vi "currentmeasure__9fa348117f.vi"() -> ()   [LabVIEW 2023]
uses:
  <instrlib>/niDCPower/nidcpower.llb/niDCPower Auto Zero.ctl
  <vilib>/Utility/error.llb/DialogType.ctl
  <instrlib>/niDCPower/nidcpower.llb/niDCPower Aperture Time Units.ctl
  <vilib>/DAQmx/read.llb/DAQmx Read (Analog 1D DBL 1Chan NSamp).vi
  <vilib>/DAQmx/create/channels.llb/DAQmx Create Channel (AI-Voltage-Basic).vi
  <vilib>/DAQmx/configure/timing.llb/DAQmx Timing (Sample Clock).vi
  <vilib>/DAQmx/configure/task.llb/DAQmx Configure Logging (TDMS).vi
  <vilib>/DAQmx/configure/trigger.llb/DAQmx Start Trigger (Digital Edge).vi
  <vilib>/DAQmx/miscellaneous.llb/DAQmx Fill In Error Info.vi
  <resource>/objmgr/daqmx.rc
panel:
  out "Waveform Graph 3":dynamicdata(graph)
  out "Waveform Graph 2":dbl[](graph)
  in  "Trigger Type":T1(tab)
  out "Waveform Graph":dbl[](graph)
  in  "Stop":bool
  in  "Number of Samples":i32=100
  in  "TDMS File Path":path
  in  "Sample Rate":dbl=1000.0
  in  "Sample Clock Source":tag="OnboardClock"
  in  "Terminal Configuration":i32(ring)=-1 items=["default"=-1, "RSE"=10083, "NRSE"=10078, "Differential"=10106, "Pseudodifferential"=12529]
  in  "Max Voltage":dbl=5.0
  in  "Min Voltage":dbl=-5.0
  in  "Physical Channel":tag="Dev1/ai0"
  out "Actual Sample Rate":dbl=1000.0 format="%0.2f"
  in  "Logging Mode":i32(ring)=10231 items=["Off"=10231, "Log and Read"=15842]
  in  "Auto Zero":T2 items=["Off"=0, "Once"=1024, "On"=1]
  in  "Measure Record Length Is Finite":bool=TRUE caption="Measure Record Length \nIs Finite"
  in  "Samples to Average":i32=1
  in  "Measure Record Length 2":i32=100 caption="Measure Record Length"
  out "Effective Measurement Rate":dbl
  in  "Voltage Level":dbl=5.0 format="%.4p"
  in  "Channel Name":string="0"
  in  "Resource Name":refnum<k15>="Dev1"
  # "To enable triggers, select a tab above, and configure the settings.\n\nNot all hardware supports all trigger types. Refer to your device documentation for more information."
  # "This trigger type is not supported in continuous sample timing. \n\nRefer to your device documentation for more information on which triggers are supported."
  # "This trigger type is not supported in continuous sample timing. \n\nRefer to your device documentation for more information on which triggers are supported."
  # "If time is not manually set, task will begin after 10 seconds"
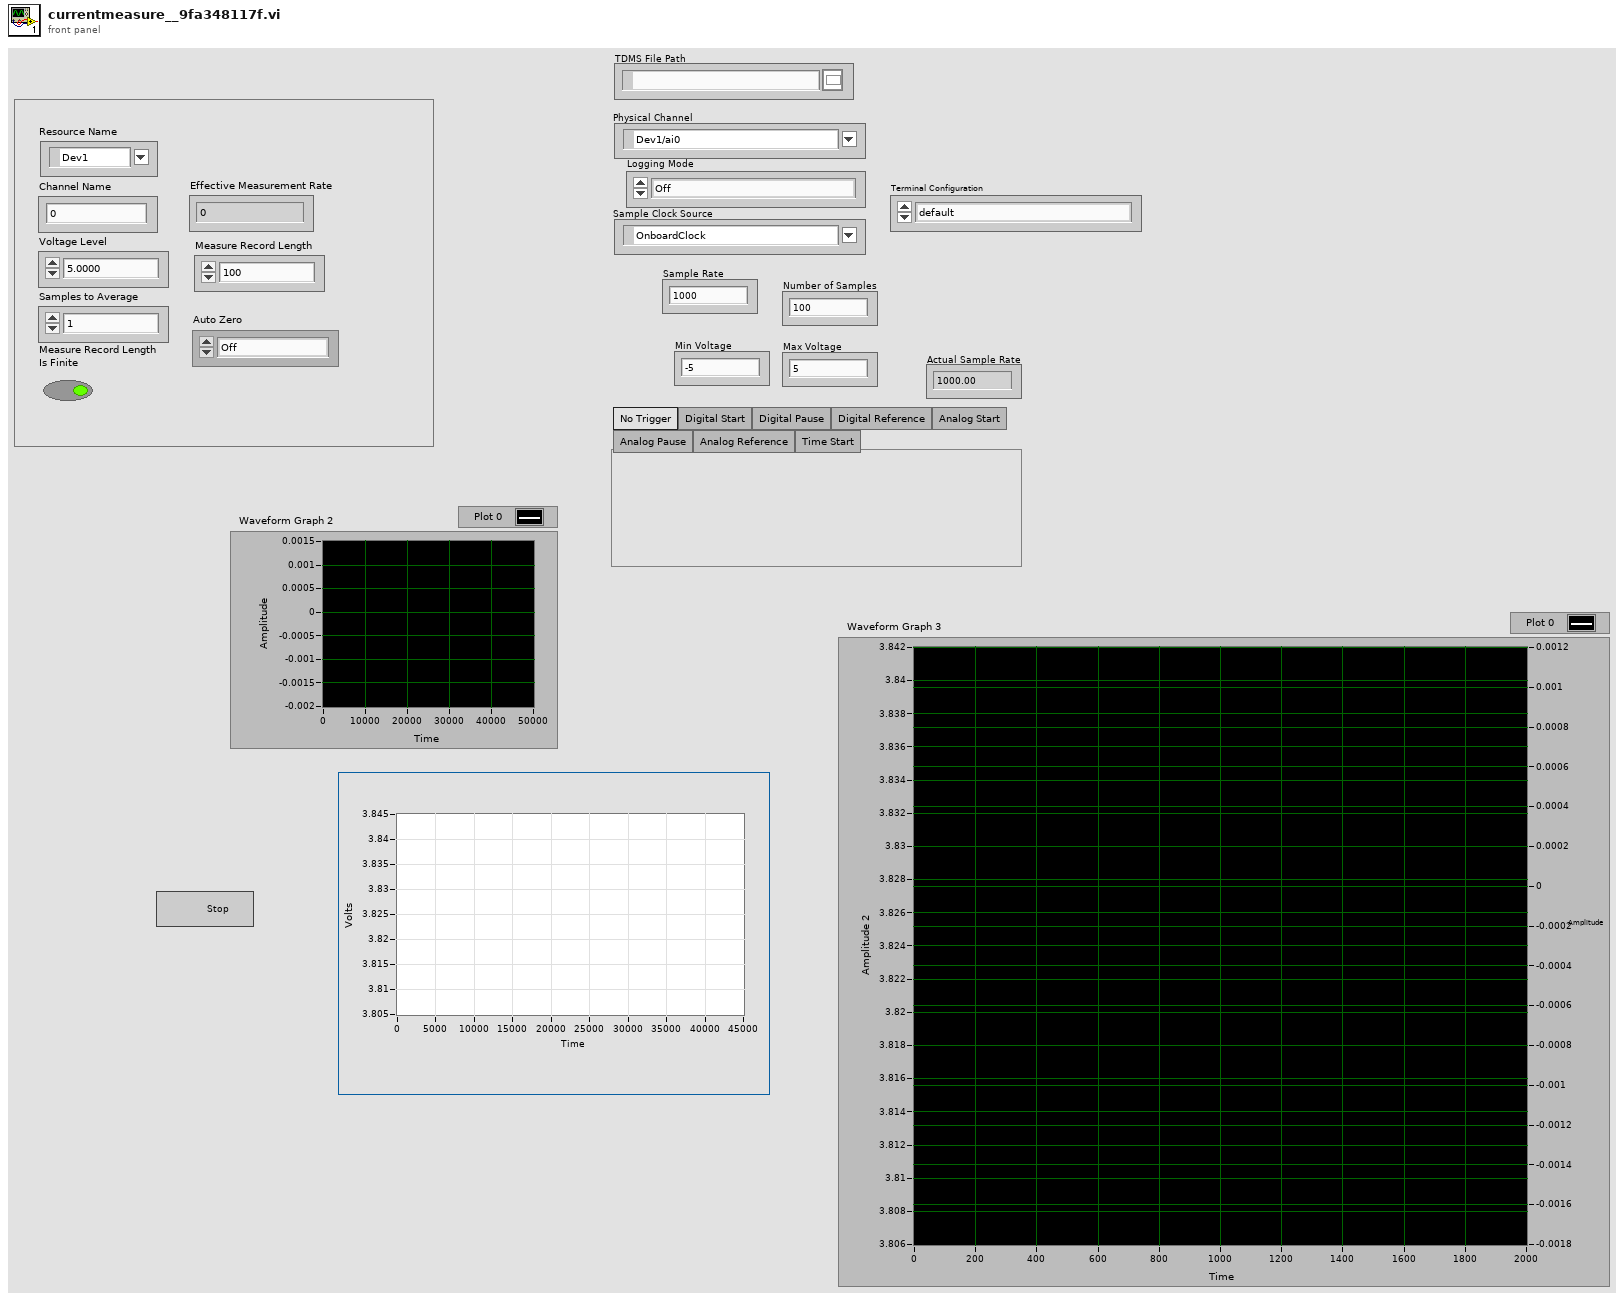
[diagram p1: front panel]
types:
  T1 = enum32{"No Trigger", "Digital Start", "Digital Pause", "Digital Reference", "Analog Start", "Analog Pause", "Analog Reference", "Time Start"}
  T2 = typedef "niDCPower Auto Zero.ctl" = i32
  T3 = typedef "DialogType.ctl" = u16
  T4 = typedef "niDCPower Aperture Time Units.ctl" = i32
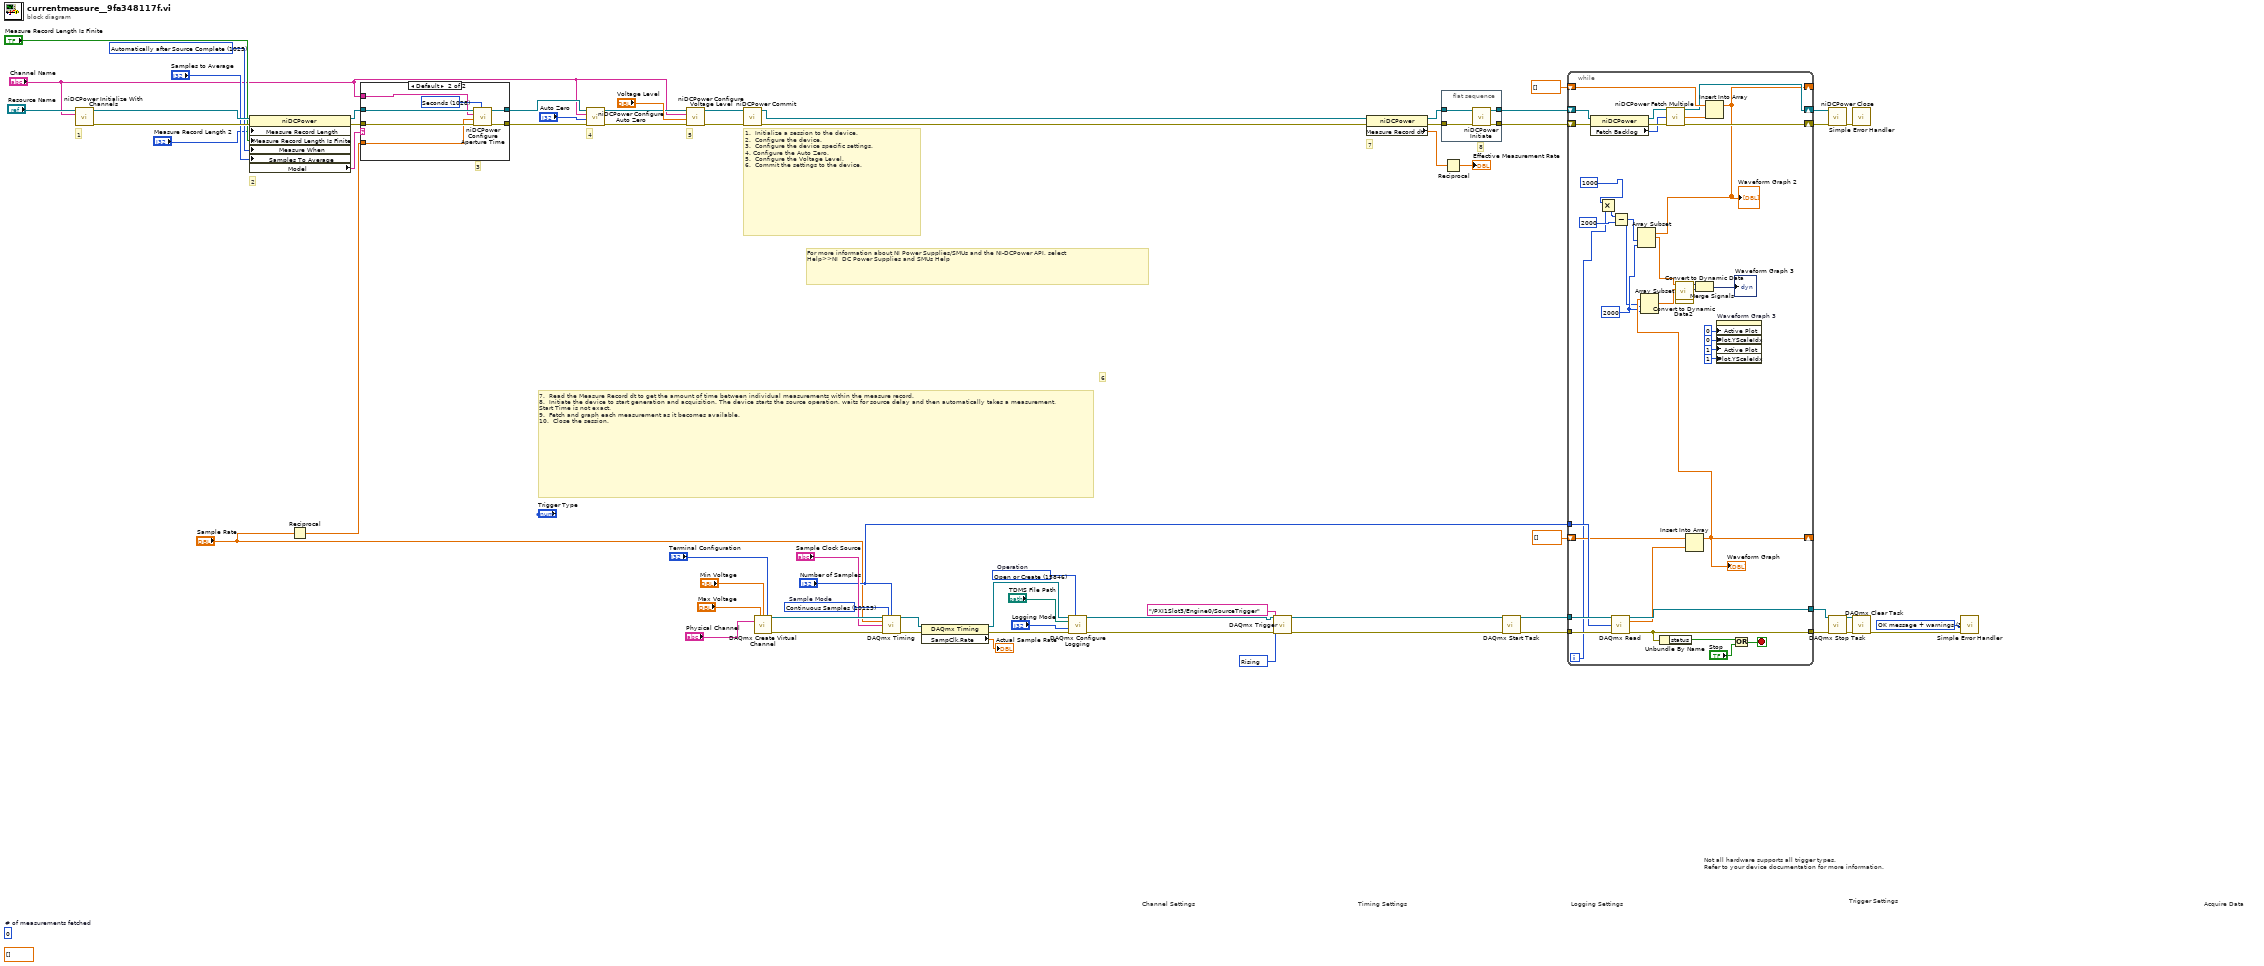
[diagram p0: block diagram]
diagram:
  w3 = 10280 items=["Rising"=10280, "Falling"=10171] ("edge")
  w19 = T3 3 items=["no dialog", "OK message", "continue or stop message", "OK message + warnings", "continue/stop + warnings"] ("type of dialog (OK msg:1)")
  w36 = 15846 items=["Open"=10437, "Open or Create"=15846, "Create or Replace"=15847, "Create"=15848]  # Operation
  w41 = 10123 items=["Finite Samples"=10178, "Continuous Samples"=10123, "Hardware Timed Single Point"=12522]  # Sample Mode
  (unwired) dbl[] []
  (unwired) 0  # # of measurements fetched
  w62 = 1025 items=["Automatically after Source Complete"=1025, "On Demand"=1026, "On Measure Trigger"=1027] ("Measurement:Advanced:Measure When")
  # "Trigger Settings"
  # "Not all hardware supports all trigger types.\nRefer to your device documentation for more information."
  # "Acquire Data"
  # "Timing Settings"
  # "Channel Settings"
  # "Logging Settings"
  # "7.  Read the Measure Record dt to get the amount of time between individual measurements within the measure record.\n8.  Initiate the device to start generation and acquisition. The device starts the source operation, waits for source delay and then automatically takes a measurement.\nStart Time is not exact.\n9.  Fetch and graph each measurement as it becomes available.\n10.  Close the session."
  # "8"
  # "7"
  # "6"
  # "5"
  # "4"
  # "2"
  # "1"
  # "1.  Initialize a session to the device.\n2.  Configure the device.\n3.  Configure the device specific settings.\n4. Configure the Auto Zero.\n5.  Configure the Voltage Level.\n6.  Commit the settings to the device."
  # "3"
  # "For more information about NI Power Supplies/SMUs and the NI-DCPower API, select\nHelp>>NI  DC Power Supplies and SMUs Help"
  n1 = call <instrlib>:"niDCPower Initialize With Channels.vi"("channels"="Channel Name", "resource name"="Resource Name") -> ("error out"=w63:errorcluster, "instrument handle out"=w64:refnum<k15>)  [unwired: 3 in, 5 out]
  n2 = property class="niDCPower"(reference=w64, error in=w63, "Measure Record Length"="Measure Record Length 2", "Measure Record Length Is Finite"="Measure Record Length Is Finite", "Measure When"=w62, "Samples To Average"="Samples to Average") -> (reference out=w53:refnum<k15>, error out=w52:errorcluster, "Model"=w54:string)
  n3 = Reciprocal(x="Sample Rate") -> (1/x=w17:dbl)
  n4 = case shown="Default" w54 {
    tunnel: w53 -> [w67 w74]
    tunnel: w52 -> [w66 w73]
    tunnel: [w66 w71] -> w50
    tunnel: [w67 w70] -> w51
    tunnel: "Channel Name" -> [_ w69]
    tunnel: w17 -> [_ w68]
    frame "NI PXI-4110", "NI PXI-4130", "NI PXI-4131A", "NI PXIe-4154" {
    }
    frame Default {
      w72 = T4 1028 items=["Seconds"=1028, "Powerline Cycles"=1029] ("aperture time units")
      n5 = call <instrlib>:"niDCPower Configure Aperture Time.vi"("aperture time units"=w72, "error in (no error)"=w73, "aperture time"=w68, "channel name"=w69, "instrument handle"=w74) -> ("error out"=w71:errorcluster, "instrument handle out"=w70:refnum<k15>)  [unwired: 5 out]
    }
  }
  n6 = call <instrlib>:"niDCPower Configure Auto Zero.vi"("error in (no error)"=w50, "auto zero"="Auto Zero", "channel name"="Channel Name", "instrument handle"=w51) -> ("error out"=w48:errorcluster, "instrument handle out"=w47:refnum<k15>)  [unwired: 6 out]
  n7 = call <instrlib>:"niDCPower Configure Voltage Level.vi"("error in (no error)"=w48, "voltage level"="Voltage Level", "channel name"="Channel Name", "instrument handle"=w47) -> ("error out"=w60:errorcluster, "instrument handle out"=w59:refnum<k15>)  [unwired: 6 out]
  n8 = call <instrlib>:"niDCPower Commit.vi"("error in (no error)"=w60, "instrument handle"=w59) -> ("error out"=w1:errorcluster, "instrument handle out"=w2:refnum<k15>)  [unwired: 8 out]
  n9 = call-poly <vilib>:"DAQmx Create Virtual Channel.vi"("maximum value"="Max Voltage", "minimum value"="Min Voltage", "input terminal configuration"="Terminal Configuration", "physical channels"="Physical Channel") -> ("task out"=w39:refnum<k21>, "error out"=w40:errorcluster)  [unwired: 10 in]
  n10 = call-poly <vilib>:"DAQmx Timing.vi"("task/channels in"=w39, "sample mode"=w41, "samples per channel"="Number of Samples", "rate"="Sample Rate", "source"="Sample Clock Source", "error in"=w40) -> ("task out"=w43:refnum<k21>, "error out"=w42:errorcluster)  [unwired: 8 in]
  n11 = property class="DAQmx Timing"(reference=w43, error in=w42) -> (reference out=w38:refnum<k21>, error out=w37:errorcluster, "SampClk.Rate"=→"Actual Sample Rate":dbl)
  n12 = call-poly <vilib>:"DAQmx Configure Logging.vi"("task/channels in"=w38, "operation"=w36, "file path"="TDMS File Path", "logging mode"="Logging Mode", "error in"=w37) -> ("task out"=w8:refnum<k21>, "error out"=w5:errorcluster)  [unwired: 9 in]
  n13 = call-poly <vilib>:"DAQmx Trigger.vi"("task/channels in"=w8, "source"=tag "/PXI1Slot3/Engine0/SourceTrigger", "edge"=w3, "error in"=w5) -> ("task out"=w7:refnum<k21>, "error out"=w6:errorcluster)  [unwired: 10 in]
  n14 = property class="niDCPower"(reference=w2, error in=w1) -> (reference out=w58:refnum<k15>, error out=w57:errorcluster, "Measure Record dt"=w45:dbl)
  n15 = flat-sequence {
    tunnel: [w78] -> w15
    tunnel: [w77] -> w16
    tunnel: w58 -> [w76]
    tunnel: w57 -> [w75]
    frame #0 {
      n16 = call <instrlib>:"niDCPower Initiate.vi"("error in (no error)"=w75, "instrument handle"=w76) -> ("error out"=w78:errorcluster, "instrument handle out"=w77:refnum<k15>)  [unwired: 8 out]
    }
  }
  n17 = Reciprocal(x=w45) -> (1/x=→"Effective Measurement Rate":dbl)
  n18 = call <vilib>:"DAQmx Start Task.vi"("task/channels in"=w7, "error in"=w6) -> ("task out"=w35:refnum<k21>, "error out"=w34:errorcluster)  [unwired: 12 in]
  n19 = while {
    tunnel: w35 -> [w114]
    tunnel: w34 -> [w113]
    tunnel: [w112] -> w23
    tunnel: [w110] -> w22
    tunnel: "Number of Samples" -> [w107]
    shift-right: [w88] -> _
    shift-left: dbl[] [] -> [w102]
    shift-right: [w100] -> w13
    shift-left: w16 -> [w106]
    shift-right: [w99] -> w12
    shift-left: w15 -> [w105]
    shift-right: [w87] -> _
    shift-left: dbl[] [] -> [w97]
    i -> [w82]
    stop <- w108 stop-if-true
    w83 = 2000 ("length")
    n20 = property class="niDCPower"(reference=w106, error in=w105) -> (reference out=w104:refnum<k15>, error out=w103:errorcluster, "Fetch Backlog"=w98:i32)
    n21 = Multiply(x=1000, y=w82) -> (x*y=w81:i32)
    n22 = call-poly <vilib>:"DAQmx Read.vi"("task/channels in"=w114, "number of samples per channel"=w107, "error in"=w113) -> ("task out"=w112:refnum<k21>, "data"=w96:dbl[], "error out"=w110:errorcluster)  [unwired: 10 in]
    n23 = Subtract(x=w81, y=2000) -> (x-y=w80:i32)
    n24 = Unbundle By Name(w110) -> ("status"=w109:bool)
    n25 = call <instrlib>:"niDCPower Fetch Multiple.vi"("instrument handle"=w104, "count (1)"=w98, "error in (no error)"=w103) -> ("instrument handle out"=w100:refnum<k15>, "current measurements"=w101:dbl[], "error out"=w99:errorcluster)  [unwired: 2 in, 8 out]
    n26 = Insert Into Array(array=w97, new element=w96) -> (w87:dbl[])  [unwired: 1 in]
    "Waveform Graph" <- w87
    n27 = Array Subset(array=w87, index=w80, length=w83) -> (w85:dbl[])
    n28 = call "Convert to Dynamic Data2"("Array"=w85) -> ("Dynamic Data Type"=w94:dynamicdata)  [unwired: 3 in]
    n29 = Insert Into Array(array=w102, new element=w101) -> (w88:dbl[])  [unwired: 1 in]
    "Waveform Graph 2" <- w88
    n30 = Array Subset(array=w88, index=w80, length=w83) -> (w86:dbl[])
    n31 = call "Convert to Dynamic Data"("Array"=w86) -> ("Dynamic Data Type"=w95:dynamicdata)  [unwired: 3 in]
    n32 = Merge Signals(w95, w94) -> (→"Waveform Graph 3":dynamicdata)
    n33 = property on="Waveform Graph 3" class="WFGraph (strict)"("Active Plot"=u32 0, "Plot.YScaleIdx"=u32 0 ("Plot.Y Scale Index"), "Active Plot"=u32 1, "Plot.YScaleIdx"=u32 1 ("Plot.Y Scale Index")) -> ()  [unwired: 2 in, 2 out]
    n34 = Or(x=w109, y="Stop") -> (x .or. y?=w108:bool)
  }
  n35 = call <instrlib>:"niDCPower Close.vi"("error in (no error)"=w12, "instrument handle"=w13) -> ("error out"=w11:errorcluster)  [unwired: 9 out]
  n36 = call <vilib>:"DAQmx Stop Task.vi"("task/channels in"=w23, "error in"=w22) -> ("task out"=w20:refnum<k21>, "error out"=w21:errorcluster)  [unwired: 12 in]
  n37 = call <vilib>:"Simple Error Handler.vi"("error in (no error)"=w11) -> ()  [unwired: 1 in, 8 out]
  n38 = call <vilib>:"DAQmx Clear Task.vi"("task in"=w20, "error in"=w21) -> ("error out"=w33:errorcluster)  [unwired: 13 in]
  n39 = call <vilib>:"Simple Error Handler.vi"("type of dialog (OK msg:1)"=w19, "error in (no error)"=w33) -> ()  [unwired: 3 in, 5 out]
